vi "VIH Dialog - VI Terminals.vi"(6 "mode (normal)":enum16{"normal", "Enum sel"}(ring), 7 "Called from Master (F)":bool, 10 "Ctrl IDs in":string[](array[string]), 11 "VI Path":path) -> (0 "OK out":bool, 1 "Ctrl Rules":T1[](array[typedef]), 2 "Ctrl IDs out":string[](array[string]), 3 "dup VI Path":path)   [LabVIEW 2014]
doc: "::: VI Helpeks :::\nCopyright (c) 2000-2026 Konstantin Shifershteyn. All rights reserved."
uses:
  _VIH HelpGen.llb/VIH HelpGen Typedef - Cluster - Control Rule.ctl
  _VIH HelpGen.llb/VIH HelpGen Typedef - Enum - Description Mode.ctl
  _VIH HelpGen.llb/VIH HelpGen Typedef - Enum - Default,Enable,Disable.ctl
  _VIH HelpGen.llb/VIH HelpGen Typedef - Cluster - Enum Value Info.ctl
  <vilib>/Utility/miscctls.llb/LVPointTypeDef.ctl
  <vilib>/event_ctls.llb/lveventtype.ctl
  <vilib>/Utility/cursorutil.llb/Set Cursor (Icon Pict).vi
  _VIH Support Library.llb/VIH Utility - APP - Is Value Changed (I32).vi
panel:
  out "Conpane Image":picture caption="Connector Pane Image"
  in  "ConpaneMenuActive":bool
  in  "Ctrl Tree":string[](tree) caption="Control Tree"
  in  "%OK":bool caption="OK"
  in  "%Cancel":bool caption="Cancel"
  # "*) use Context Help for information on the controls"
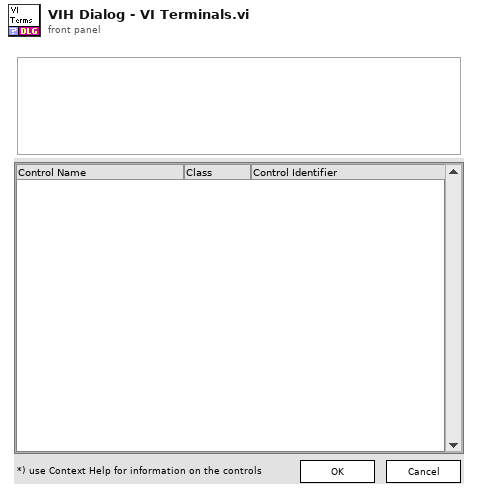
[diagram p1: front panel]
types:
  T1 = typedef "VIH HelpGen Typedef - Cluster - Control Rule.ctl" = cluster{"CtrlID":string, "CustomRule":bool, "DscrMode":T2, "Description":string, "ClusterMembers":T3, "EnumValues":T3, "EnumValDscr":T4[], "CustomName":string}
  T2 = typedef "VIH HelpGen Typedef - Enum - Description Mode.ctl" = enum16{"Default", "Description", "Description1", "Description2", "Custom", "None"}
  T3 = typedef "VIH HelpGen Typedef - Enum - Default,Enable,Disable.ctl" = enum16{"Default", "Enable", "Disable"}
  T4 = typedef "VIH HelpGen Typedef - Cluster - Enum Value Info.ctl" = cluster{"Value":ext, "String":string, "Description":string}
  T5 = typedef "LVPointTypeDef.ctl" = cluster{"Horizontal":i16, "Vertical":i16}
  T6 = typedef "lveventtype.ctl" = enum32{"Null", "Timeout", "Annotation Menu Selection", "Annotation Menu Selection?", "App Instance Close", "App Instance Close?", "Autoscale Range Change", "Bookmark Info Change", "Cell Edit", "Cell Edit?", "Cursor Grab", "Cursor Grab?", "Cursor Menu Selection", "Cursor Menu Selection?", "Cursor Move", "Cursor Release", "Data Change", "Direction Change", "Display State Change", "Drag Ended", "Drag Enter", "Drag Leave", "Drag Over", "Drag Source Update", "Drag Starting", "Drag Starting?", "Drop", "Exec State Change", "Key Down", "Key Down?", "Key Repeat", "Key Repeat?", "Key Up", "Listbox Double Click", "Menu Activation?", "Menu Selection (App)", "Menu Selection? (App)", "Menu Selection (User)", "Mouse Down", "Mouse Down?", "Mouse Enter", "Mouse Leave", "Mouse Move", "Mouse Up", "Mouse Wheel", "NI Security User Change (App)", "Pane Size", "Panel Close", "Panel Close?", "Panel Resize", "Plot Attribute Change", "Scale Range Change", "Shortcut Menu Activation?", "Shortcut Menu Selection (App)", "Shortcut Menu Selection? (App)", "Shortcut Menu Selection (User)", "Tree Double Click", "Tree Drag", "Tree Drag?", "Tree Drop", "Tree Drop?", "Tree Item Close", "Tree Item Close?", "Tree Item Open", "Tree Item Open?", "User Event", "Value Change"}
  T7 = cluster{"Width":i16, "Style":enum32{"Solid", "Dash", "Dot", "DashDot", "DashDotDot"}}
  T8 = typedef "LVPoint32TypeDef.ctl" = cluster{"Horizontal":i32, "Vertical":i32}
  T9 = typedef "LVMouseTypeDef.ctl" = cluster{"Mouse Position":cluster{"X":i32, "Y":i32}, "Mouse Modifiers":cluster{"Button Down":bool, "Shift Mod":bool, "Menu Mod":bool, "Option Mod":bool}}
  T10 = cluster{"Button Down":bool, "Shift Mod":bool, "Menu Mod":bool, "Option Mod":bool}
  T11 = cluster{"Ctrl ID":string, "Conpane Idx":i32, "Bounds":cluster{"X0":i32, "Y0":i32, "X1":i32, "Y1":i32}}[]
  T12 = cluster{"Ctrl ID":string, "Conpane Idx":i32, "Bounds":cluster{"X0":i32, "Y0":i32, "X1":i32, "Y1":i32}}
  T13 = typedef "VIH Project Tree Typedef - Tree Refnum.ctl" = refnum<vi>
  T14 = cluster{"Control Label":string, "Class Name":string, "Indicator":bool, "Error Cluster":bool, "Tree Tag":string, "Control ID":string, "Conpane Idx":i32}
  T15 = typedef "imagedata.ctl" = cluster{"image type":i32, "image depth":i32, "image":u8[], "mask":u8[], "colors":u32[], "Rectangle":cluster{"left":i16, "top":i16, "right":i16, "bottom":i16}}
  T16 = cluster{"left":i16, "top":i16, "right":i16, "bottom":i16}
  T17 = typedef "VIH HelpGen Typedef - Control Terminal Attributes Cluster.ctl" = cluster{"Conpane Idx":i32, "Control":bool, "Wire Rule":enum16{"Invalid Wire Rule", "Required", "Recommended", "Optional", "Dynamic Dispatch"}}
  T18 = cluster{"Control Label":string, "Class Name":string, "Indicator":bool, "Error Cluster":bool, "Tree Tag":string, "Control ID":string, "Conpane Idx":i32}[]
  T19 = typedef "LVBoundsTypeDef.ctl" = cluster{"Width":u32, "Height":u32}
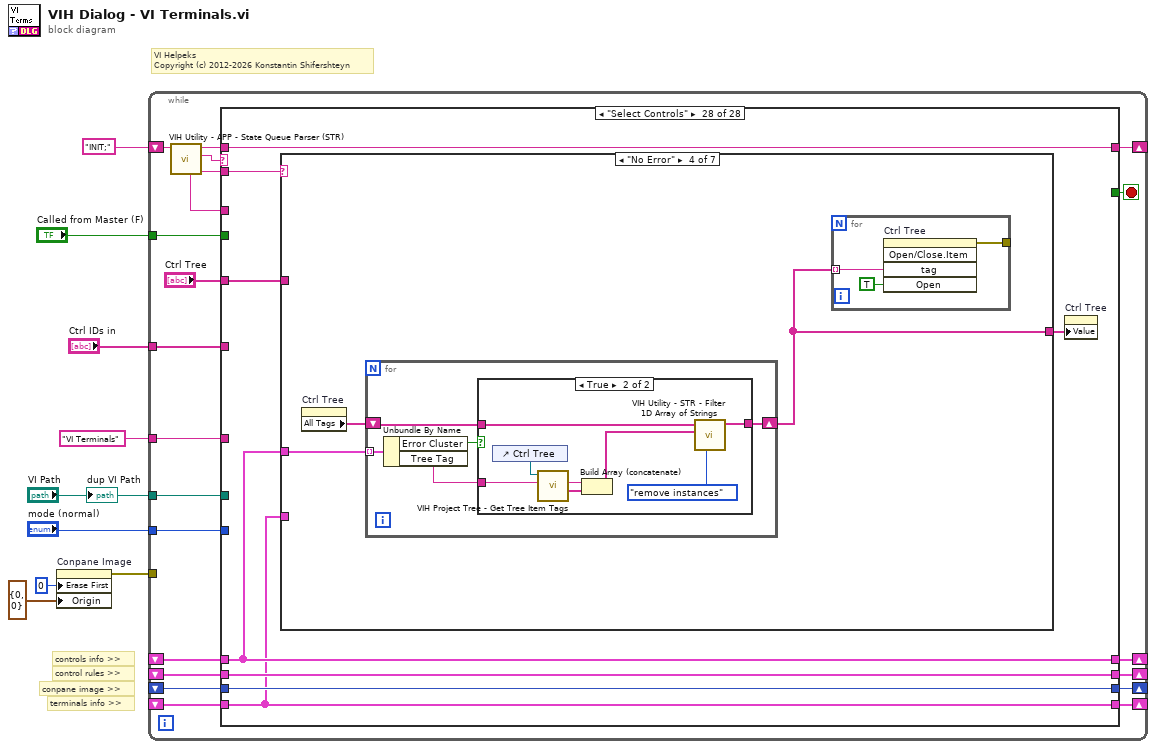
[diagram p0: block diagram]
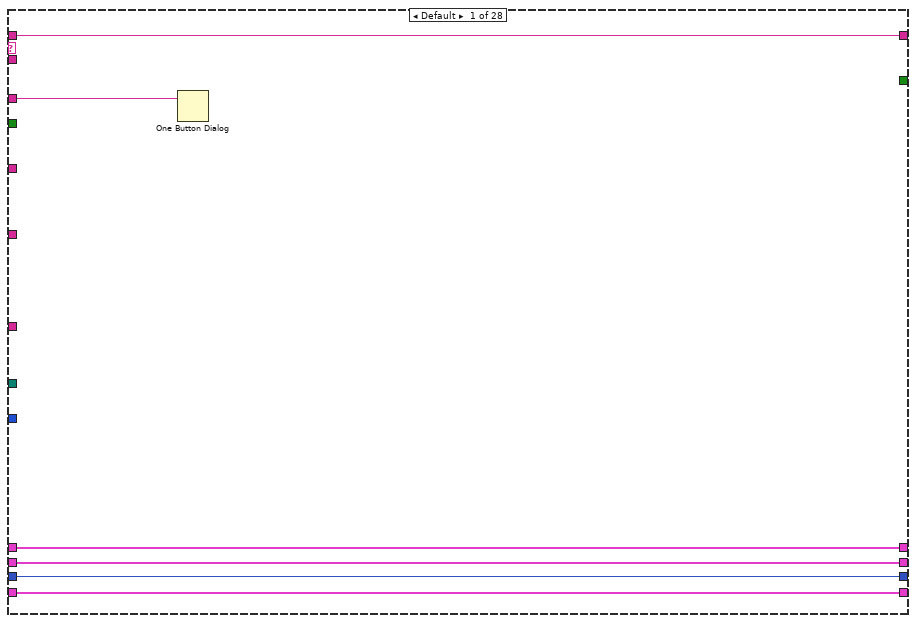
[diagram p2: hidden frame]
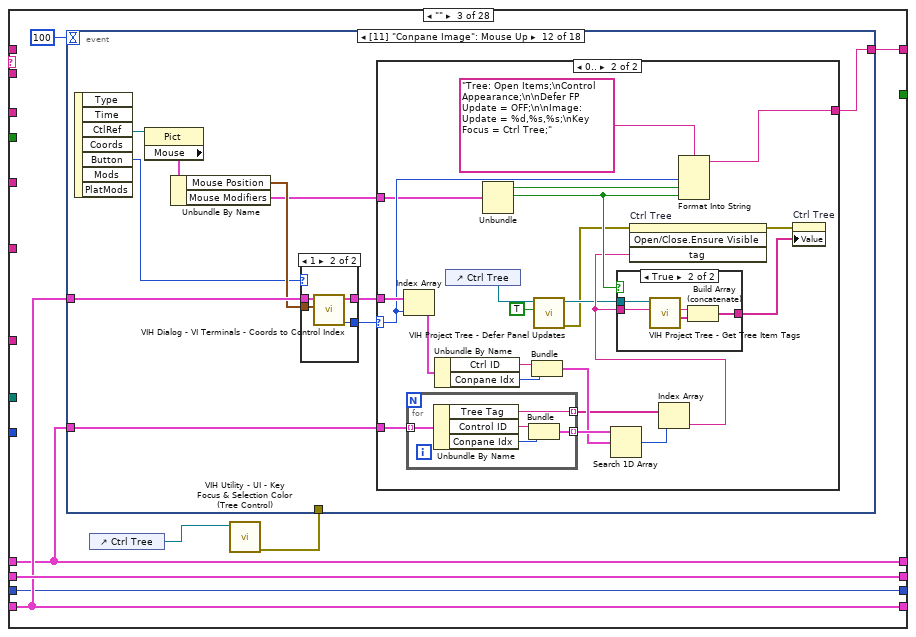
[diagram p4: hidden frame]
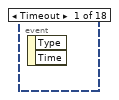
[diagram p5: hidden frame]
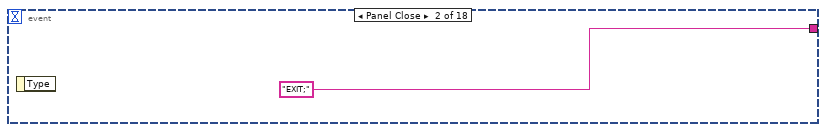
[diagram p6: hidden frame]
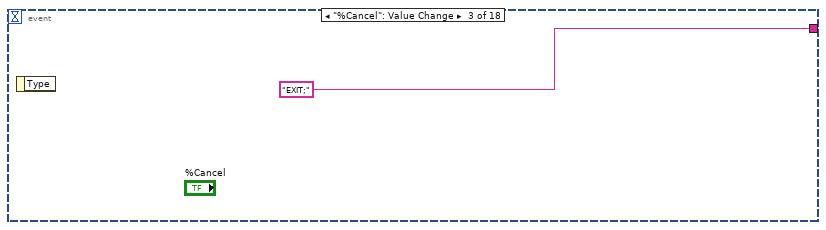
[diagram p7: hidden frame]
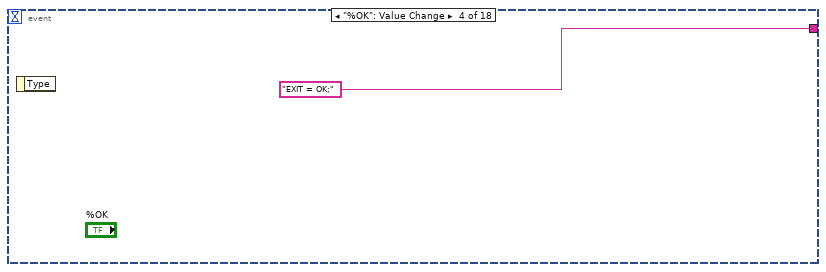
[diagram p8: hidden frame]
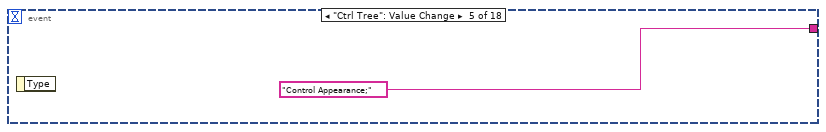
[diagram p9: hidden frame]
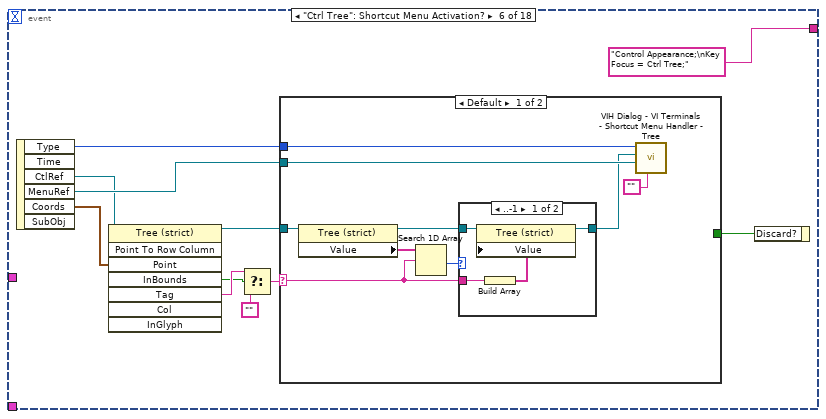
[diagram p10: hidden frame]
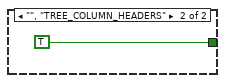
[diagram p12: hidden frame]
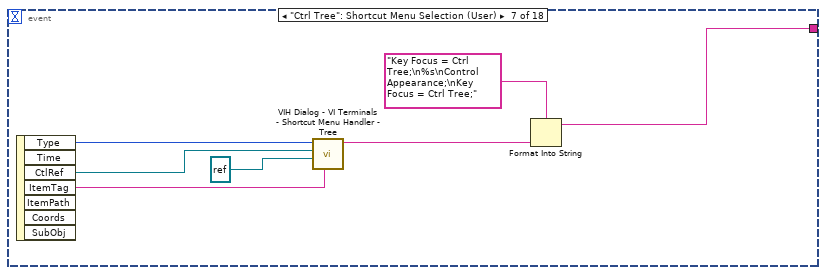
[diagram p13: hidden frame]
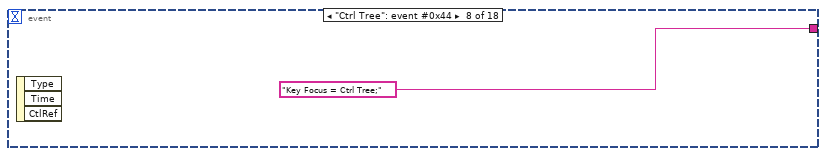
[diagram p14: hidden frame]
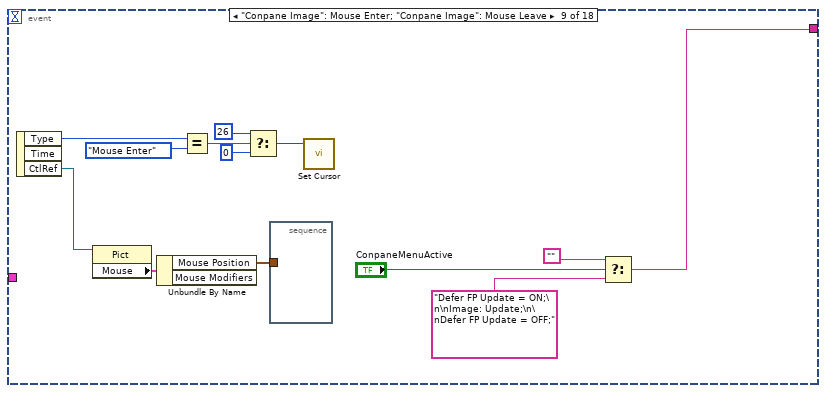
[diagram p15: hidden frame]
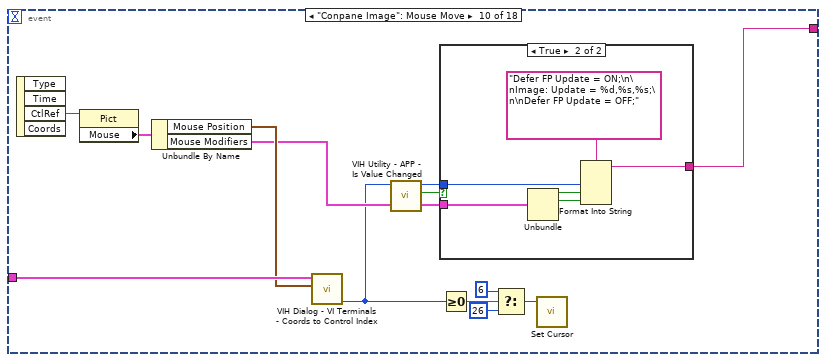
[diagram p16: hidden frame]
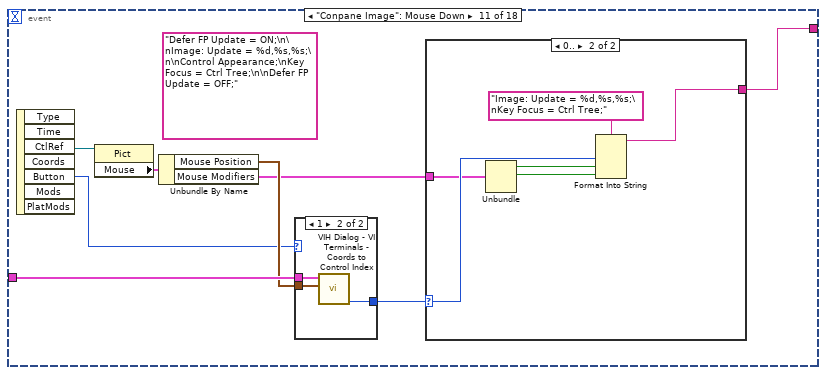
[diagram p18: hidden frame]
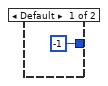
[diagram p19: hidden frame]
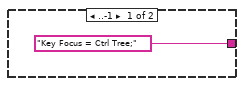
[diagram p20: hidden frame]
diagram:
  # "VI Helpeks\nCopyright (c) 2012-2026 Konstantin Shifershteyn"
  # "terminals info >>"
  # "conpane image >>"
  # "controls info >>"
  # "control rules >>"
  n1 = property on="Conpane Image" class="Pict"("Erase First"=u8 0, "Origin"=T5 {"Horizontal"=0, "Vertical"=0}) -> (error out=w5:errorcluster)  [unwired: 2 in, 1 out]
  n2 = while {
    shift-right: [w27] -> _
    shift-left: "INIT;" -> [w29]
    tunnel: "VI Path" -> [w25]
    shift-right: [w21] -> _
    shift-left: _ -> [w20]
    shift-right: [w19] -> _
    shift-left: _ -> [w18]
    shift-right: [w17] -> _
    shift-left: _ -> [w16]
    tunnel: w5 -> [_]
    tunnel: "Ctrl IDs in" -> [w15]
    tunnel: "mode (normal)" -> [w14]
    tunnel: "Called from Master (F)" -> [w13]
    shift-right: [w12] -> _
    shift-left: _ -> [w11]
    tunnel: "VI Terminals" -> [w10]
    stop <- w22 stop-if-true
    n3 = call "VIH Utility - APP - State Queue Parser (STR).vi"("input queue"=w29) -> ("state parameters"=w24:string, "state"=w30:string, "remained queue"=w28:string, "complete state specifier"=w26:string)  [unwired: 5 in]
    n4 = case shown="\"Select Controls\"" w30 {
      tunnel: w28 -> [w36 w41 _ w286 _ w327 w332 w338 w346 w359 w383 w389 w394 w439 w452 w491 w504 w510 w516 w523 w537 w569 w578 w595 w616 w639 w646 w654]
      tunnel: [w36 w41 w46 w280 "Tree: Reset;\nHALT;" w327 w332 w338 w346 w359 w383 w389 w394 w439 w452 w491 w504 w510 w516 w523 w537 w569 w578 w595 w616 w639 w646 w654] -> w27
      tunnel: w26 -> [w35 _ _ _ _ _ _ _ _ _ _ _ _ _ _ _ _ _ _ _ _ _ _ _ _ _ _ _]
      tunnel: w25 -> [_ _ _ _ _ _ _ _ _ _ _ _ _ w438 _ _ _ _ _ _ _ _ _ _ _ _ _ _]
      tunnel: w24 -> [_ _ _ _ w293 _ _ w337 w345 _ w380 _ _ _ _ _ _ _ _ _ w535 _ _ _ _ _ _ w651]
      tunnel: "Ctrl Tree" -> [_ _ _ _ w292 _ _ _ _ w353 _ _ _ _ _ _ _ _ w512 _ _ _ w581 w598 w609 w635 _ w650]
      tunnel: [_ _ _ _ _ TRUE _ _ _ _ _ _ _ _ _ _ _ _ _ _ _ _ _ _ _ _ _ _] -> w22
      tunnel: [w34 w40 w45 w283 w291 w325 w331 w336 w342 w354 w382 w388 w393 w434 w447 w487 T1[] [] w508 w515 w522 w536 w568 w580 w597 w617 w631 w645 w648] -> w21
      tunnel: w20 -> [w34 w40 w45 w283 w291 w325 w331 w336 w342 w354 w382 w388 w393 _ w447 w487 _ w508 w515 w522 w536 w568 w580 w597 w617 w631 w645 w648]
      tunnel: [w33 w39 w44 w282 w290 w323 w330 w335 w341 w358 w381 w387 w392 w417 w445 w489 w501 w507 w514 w521 w531 w567 w572 w593 w614 w637 w644 w647] -> w19
      tunnel: w18 -> [w33 w39 w44 w282 w290 w323 w330 w335 w341 w358 w381 w387 w392 _ w445 w489 w501 w507 w514 w521 w531 w567 w572 w593 w614 w637 w644 w647]
      tunnel: [w32 w38 w43 w281 w289 w322 w329 w334 w340 w357 w379 w386 w391 w404 w446 w490 w500 w506 w513 w520 w530 w566 w571 w592 w613 w636 w643 w653] -> w17
      tunnel: w16 -> [w32 w38 w43 w281 w289 w322 w329 w334 w340 w357 w379 w386 w391 _ w446 w490 w500 w506 w513 w520 w530 w566 w571 w592 w613 w636 w643 w653]
      tunnel: w15 -> [_ _ _ _ _ _ _ _ _ _ _ _ _ _ w450 _ _ _ _ _ _ _ _ _ _ _ _ _]
      tunnel: w14 -> [_ _ _ w271 _ _ _ _ _ w356 _ _ _ _ _ _ _ _ _ _ _ _ _ _ _ _ _ _]
      tunnel: w13 -> [_ _ _ w273 _ _ _ _ _ w351 _ _ _ _ w448 _ _ _ _ _ _ _ _ _ _ _ _ _]
      tunnel: [w31 w37 w42 w274 w288 w321 w328 w333 w339 w348 w378 w385 w390 w396 w444 w488 w499 w505 w511 w519 w524 w565 w570 w589 w611 w626 w642 w649] -> w12
      tunnel: w11 -> [w31 w37 w42 w274 w288 w321 w328 w333 w339 w348 w378 w385 w390 _ w444 w488 w499 w505 w511 w519 w524 w565 w570 w589 w611 w626 w642 w649]
      tunnel: w10 -> [_ _ _ w268 _ w316 _ _ _ _ _ _ _ _ _ _ _ _ _ _ _ _ _ _ _ _ _ _]
      frame Default {
        n5 = One Button Dialog(message=w35) -> ()  [unwired: 1 in, 1 out]
      }
      frame "#" {
      }
      frame "" {
        n6 = control-ref of="Ctrl Tree"() -> (w48:refnum<vi>)
        n7 = call "VIH Utility - UI - Key Focus & Selection Color (Tree Control).vi"("Tree Refnum"=w48) -> ("error out"=w47:errorcluster)  [unwired: 8 in, 2 out]
        n8 = event shown="[11] \"Conpane Image\": Mouse Up" {
          selector: _ -> [_ _ _ _ _ _ _ _ _ _ _ _ _ _ _ _ _ _]
          dyn-events: _ -> [_ _ _ _ _ _ _ _ _ _ _ _ _ _ _ _ _ _]
          timeout: 100 -> [_ _ _ _ _ _ _ _ _ _ _ _ _ _ _ _ _ _]
          tunnel: w47 -> [_ _ _ _ _ _ _ _ _ _ _ _ _ _ _ _ _ _]
          tunnel: [_ "EXIT;" "EXIT;" "EXIT = OK;" "Control Appearance;" "Control Appearance;\nKey Focus = Ctrl Tree;" w81 "Key Focus = Ctrl Tree;" w91 w109 w125 w145 w208 w236 "Key Focus = Ctrl Tree;" "Image: Update;" "Image: Update;" w260] -> w46
          tunnel: w44 -> [_ _ _ _ _ _ _ _ _ w113 w127 w148 w214 w233 w248 _ _ w261]
          tunnel: w42 -> [_ _ _ _ _ _ _ _ _ _ _ w139 w192 w220 _ _ _ _]
          event Timeout {
            n9 = event-data() -> ()  [unwired: 1 in, 2 out]
          }
          event Panel Close {
            n10 = event-data() -> ()  [unwired: 1 in, 1 out]
          }
          event "%Cancel": Value Change {
            n11 = event-data() -> ()  [unwired: 1 in, 1 out]
          }
          event "%OK": Value Change {
            n12 = event-data() -> ()  [unwired: 1 in, 1 out]
          }
          event "Ctrl Tree": Value Change {
            n13 = event-data() -> ()  [unwired: 1 in, 1 out]
          }
          event "Ctrl Tree": Shortcut Menu Activation? {
            n14 = event-data() -> ("Type"=w57:T6, "CtlRef"=w54:refnum<vi>, "MenuRef"=w56:refnum<k9>, "Coords"=w55:T8)  [unwired: 1 in, 2 out]
            n15 = invoke class="Tree (strict)" method="Point To Row Column"(reference=w54, "Point"=w55) -> (reference out=w63:refnum<vi>, "InBounds"=w59:bool, "Tag"=w60:string)  [unwired: 6 in, 5 out]
            n16 = Select(t=w60, s=w59, f="") -> (s? t:f=w62:string)
            n17 = case shown="Default" w62 {
              selector: w62 -> [w68 _]
              tunnel: w56 -> [w69 _]
              tunnel: [_ TRUE] -> w58
              tunnel: w63 -> [w66 _]
              tunnel: w57 -> [w70 _]
              frame Default {
                n18 = property class="Tree (strict)"(reference=w66) -> (reference out=w71:refnum<vi>, "Value"=w73:string[])  [unwired: 1 in, 1 out]
                n19 = Search 1D Array(1D array=w73, element=w68) -> (index of element=w72:i32)  [unwired: 1 in]
                n20 = case shown="..-1" w72 {
                  tunnel: w71 -> [w77 w78]
                  tunnel: w68 -> [w76 _]
                  tunnel: [w74 w78] -> w65
                  frame ..-1 {
                    n21 = Build Array(w76) -> (w75:string[])
                    n22 = property class="Tree (strict)"(reference=w77, "Value"=w75) -> (reference out=w74:refnum<vi>)  [unwired: 1 in, 1 out]
                  }
                  frame 0.. {
                  }
                }
                n23 = call "VIH Dialog - VI Terminals - Shortcut Menu Handler - Tree.vi"("Menu Tag"="", "MenuRef"=w69, "Terminals Tree"=w65, "Event Type"=w70) -> ()  [unwired: 7 in, 1 out]
              }
              frame "", "TREE_COLUMN_HEADERS" {
              }
            }
            n24 = event-data("Discard?"=w58) -> ()  [unwired: 1 in, 1 out]
          }
          event "Ctrl Tree": Shortcut Menu Selection (User) {
            n25 = event-data() -> ("Type"=w85:T6, "CtlRef"=w84:refnum<vi>, "ItemTag"=w83:string)  [unwired: 1 in, 4 out]
            n26 = call "VIH Dialog - VI Terminals - Shortcut Menu Handler - Tree.vi"("Menu Tag"=w83, "MenuRef"=refnum<k9> refnum, "Terminals Tree"=w84, "Event Type"=w85) -> ("States spec"=w82:string)  [unwired: 7 in]
            n27 = Format Into String(format string="Key Focus = Ctrl Tree;\n%s\nControl Appearance;\nKey Focus = Ctrl Tree;", w82) -> (resulting string=w81:string)  [unwired: 2 in, 1 out]
          }
          event "Ctrl Tree": event #0x44 {
            n28 = event-data() -> ()  [unwired: 1 in, 3 out]
          }
          event "Conpane Image": Mouse Enter; "Conpane Image": Mouse Leave {
            n29 = event-data() -> ("Type"=w100:T6, "CtlRef"=w89:refnum<vi>)  [unwired: 1 in, 1 out]
            n30 = property on="Property Node" class="Pict"(reference=w89) -> ("Mouse"=w90:T9)  [unwired: 1 in, 2 out]
            n31 = Unbundle By Name(w90) -> ("Mouse Position"=w88:cluster{"X":i32, "Y":i32})  [unwired: 1 out]
            n32 = Equal?(x=w100, y=lveventtype."Mouse Enter" ("Type")) -> (x = y?=w98:bool)
            n33 = Select(t=u16 26 ("icon"), s=w98, f=u16 0) -> (s? t:f=w95:u16)
            n34 = stacked-sequence {
              tunnel: w88 -> [_]
              frame #0 {
              }
            }
            n35 = call-poly <vilib>:"Set Cursor.vi"("icon"=w95) -> ()  [unwired: 9 in, 2 out]
            n36 = Select(t="", s="ConpaneMenuActive", f="Defer FP Update = ON;\n\nImage: Update;\n\nDefer FP Update = OFF;") -> (s? t:f=w91:string)
          }
          event "Conpane Image": Mouse Move {
            n37 = event-data() -> ("CtlRef"=w112:refnum<vi>)  [unwired: 1 in, 3 out]
            n38 = property on="Property Node" class="Pict"(reference=w112) -> ("Mouse"=w111:T9)  [unwired: 1 in, 2 out]
            n39 = Unbundle By Name(w111) -> ("Mouse Position"=w110:cluster{"X":i32, "Y":i32}, "Mouse Modifiers"=w106:T10)
            n40 = call "VIH Dialog - VI Terminals - Coords to Control Index.vi"("Coords"=w110, "Controls info"=w113) -> ("Index"=w101:i32)  [unwired: 8 in, 1 out]
            n41 = call-poly "VIH Utility - APP - Is Value Changed.vi"("Value"=w101) -> ("Changed"=w107:bool, "dup Value"=w108:i32)  [unwired: 5 in]
            n42 = case shown="True" w107 {
              tunnel: [_ w118] -> w109
              tunnel: w108 -> [_ w117]
              tunnel: w106 -> [_ w116]
              frame False {
              }
              frame True {
                n43 = Unbundle(w116) -> ("Button Down"=w115:bool, "Shift Mod"=w114:bool)  [unwired: 2 out]
                n44 = Format Into String(format string="Defer FP Update = ON;\n\nImage: Update = %d,%s,%s;\n\nDefer FP Update = OFF;", w117, w115, w114) -> (resulting string=w118:string)  [unwired: 2 in, 1 out]
              }
            }
            n45 = Greater Or Equal To 0?(x=w101) -> (x >= 0?=w105:bool)
            n46 = Select(t=u16 6 ("icon"), s=w105, f=u16 26) -> (s? t:f=w104:u16)
            n47 = call-poly <vilib>:"Set Cursor.vi"("icon"=w104) -> ()  [unwired: 9 in, 2 out]
          }
          event "Conpane Image": Mouse Down {
            (unwired) "Defer FP Update = ON;\n\nImage: Update = %d,%s,%s;\n\nControl Appearance;\nKey Focus = Ctrl Tree;\n\nDefer FP Update = OFF;"
            n48 = event-data() -> ("CtlRef"=w123:refnum<vi>, "Button"=w120:u16)  [unwired: 1 in, 5 out]
            n49 = property on="Property Node" class="Pict"(reference=w123) -> ("Mouse"=w124:T9)  [unwired: 1 in, 2 out]
            n50 = Unbundle By Name(w124) -> ("Mouse Position"=w122:cluster{"X":i32, "Y":i32}, "Mouse Modifiers"=w121:T10)
            n51 = case shown="1" w120 {
              tunnel: w127 -> [_ w131]
              tunnel: [-1 ("Index") w130] -> w126
              tunnel: w122 -> [_ w129]
              frame Default {
              }
              frame 1 {
                n52 = call "VIH Dialog - VI Terminals - Coords to Control Index.vi"("Coords"=w129, "Controls info"=w131) -> ("Index"=w130:i32)  [unwired: 8 in, 1 out]
              }
            }
            n53 = case shown="0.." w126 {
              selector: w126 -> [_ w137]
              tunnel: ["Key Focus = Ctrl Tree;" w136] -> w125
              tunnel: w121 -> [_ w134]
              frame ..-1 {
              }
              frame 0.. {
                n54 = Unbundle(w134) -> ("Button Down"=w133:bool, "Shift Mod"=w135:bool)  [unwired: 2 out]
                n55 = Format Into String(format string="Image: Update = %d,%s,%s;\nKey Focus = Ctrl Tree;", w137, w133, w135) -> (resulting string=w136:string)  [unwired: 2 in, 1 out]
              }
            }
          }
          event "Conpane Image": Mouse Up {
            n56 = event-data() -> ("CtlRef"=w143:refnum<vi>, "Button"=w140:u16)  [unwired: 1 in, 5 out]
            n57 = property on="Property Node" class="Pict"(reference=w143) -> ("Mouse"=w144:T9)  [unwired: 1 in, 2 out]
            n58 = Unbundle By Name(w144) -> ("Mouse Position"=w142:cluster{"X":i32, "Y":i32}, "Mouse Modifiers"=w141:T10)
            n59 = case shown="1" w140 {
              tunnel: w148 -> [w150 w154]
              tunnel: [w150 w153] -> w147
              tunnel: [-1 ("Index") w152] -> w146
              tunnel: w142 -> [_ w151]
              frame 0, Default {
              }
              frame 1 {
                n60 = call "VIH Dialog - VI Terminals - Coords to Control Index.vi"("Coords"=w151, "Controls info"=w154) -> ("Index"=w152:i32, "dup Controls info"=w153:T11)  [unwired: 8 in]
              }
            }
            n61 = case shown="0.." w146 {
              selector: w146 -> [_ w174]
              tunnel: w147 -> [_ w177]
              tunnel: ["Key Focus = Ctrl Tree;" w173] -> w145
              tunnel: w141 -> [_ w172]
              tunnel: w139 -> [_ w167]
              frame ..-1 {
                (unwired) "Image: Update;\nKey Focus = Ctrl Tree;"
              }
              frame 0.. {
                n62 = Index Array(array=w177, index=w174) -> (element=w176:T12)
                n63 = for {
                  tunnel: w167 -> [w182] mode=indexing
                  tunnel: [w180] -> w166 mode=indexing
                  tunnel: [w179] -> w162 mode=indexing
                  n64 = Unbundle By Name(w182) -> ("Tree Tag"=w179:string, "Control ID"=w181:string, "Conpane Idx"=w178:i32)
                  n65 = Bundle("Control ID"=w181, "Conpane Idx"=w178) -> (w180:cluster{"Control ID":string, "Conpane Idx":i32})  [unwired: 1 in]
                }
                n66 = Unbundle By Name(w176) -> ("Ctrl ID"=w165:string, "Conpane Idx"=w164:i32)
                n67 = control-ref of="Ctrl Tree"() -> (w157:refnum<vi>)
                n68 = Unbundle(w172) -> ("Button Down"=w171:bool, "Shift Mod"=w168:bool)  [unwired: 2 out]
                n69 = Bundle("Ctrl ID"=w165, "Conpane Idx"=w164) -> (w163:cluster{"Ctrl ID":string, "Conpane Idx":i32})  [unwired: 1 in]
                n70 = call "VIH Project Tree - Defer Panel Updates.vi"("Defer Panel Updates (F)"=TRUE, "Project Tree"=w157) -> ("error out"=w156:errorcluster, "dup Project Tree"=w158:T13)  [unwired: 7 in, 1 out]
                n71 = Search 1D Array(1D array=w166, element=w163) -> (index of element=w161:i32)  [unwired: 1 in]
                n72 = Index Array(array=w162, index=w161) -> (element=w160:string)
                n73 = case shown="True" w168 {
                  tunnel: [w183 w189] -> w170
                  tunnel: w158 -> [_ w188]
                  tunnel: w160 -> [w184 w187]
                  frame False {
                    n74 = Build Array(w184) -> (w183:string[])
                  }
                  frame True {
                    n75 = call "VIH Project Tree - Get Tree Item Tags.vi"("Parent Item Tag"=w187, "Project Tree"=w188) -> ("Child Item Tags"=w185:string[], "dup Parent Item Tag"=w186:string)  [unwired: 6 in, 2 out]
                    n76 = Build Array (concatenate)(w186, w185) -> (w189:string[])
                  }
                }
                n77 = invoke on="Ctrl Tree" class="Tree (strict)" method="Open/Close.Ensure Visible"(error in=w156, "tag"=w160) -> (error out=w169:errorcluster)  [unwired: 2 in, 3 out]
                n78 = Format Into String(format string="Tree: Open Items;\nControl Appearance;\n\nDefer FP Update = OFF;\n\nImage: Update = %d,%s,%s;\nKey Focus = Ctrl Tree;", w174, w171, w168) -> (resulting string=w173:string)  [unwired: 2 in, 1 out]
                n79 = property on="Ctrl Tree" class="Tree (strict)"(error in=w169, "Value"=w170) -> ()  [unwired: 1 in, 2 out]
              }
            }
          }
          event "Conpane Image": Shortcut Menu Activation? {
            n80 = event-data() -> ("Type"=w211:T6, "CtlRef"=w202:refnum<vi>, "MenuRef"=w209:refnum<k9>, "Coords"=w201:T8)  [unwired: 1 in, 1 out]
            n81 = local write "ConpaneMenuActive"(TRUE ("ConpaneMenuActive")) -> ()
            n82 = call "VIH UI - Convert Pane Coords to Picture Control Coords.vi"("Pane Coords"=w201, "Pict Refnum"=w202) -> ("Picture Coords"=w200:cluster{"Horizontal":i32, "Vertical":i32})  [unwired: 8 in, 1 out]
            n83 = call "VIH Dialog - VI Terminals - Coords to Control Index.vi"("Coords"=w200, "Controls info"=w214) -> ("Index"=w213:i32, "dup Controls info"=w212:T11)  [unwired: 8 in]
            n84 = for {
              tunnel: w192 -> [w218] mode=indexing
              tunnel: [w216] -> w196 mode=indexing
              n85 = Unbundle By Name(w218) -> ("Control ID"=w217:string, "Conpane Idx"=w215:i32)
              n86 = Bundle("Control ID"=w217, "Conpane Idx"=w215) -> (w216:cluster{"Control ID":string, "Conpane Idx":i32})  [unwired: 1 in]
            }
            n87 = Index Array(array=w212, index=w213) -> (element=w191:T12)
            n88 = Unbundle By Name(w191) -> ("Ctrl ID"=w195:string, "Conpane Idx"=w194:i32)
            n89 = Bundle("Ctrl ID"=w195, "Conpane Idx"=w194) -> (w193:cluster{"Ctrl ID":string, "Conpane Idx":i32})  [unwired: 1 in]
            n90 = control-ref of="Ctrl Tree"() -> (w210:refnum<vi>)
            n91 = Search 1D Array(1D array=w196, element=w193) -> (index of element=w190:i32)  [unwired: 1 in]
            n92 = Index Array(array=w192, index=w190) -> (element=w199:T14)
            n93 = Unbundle By Name(w199) -> ("Tree Tag"=w197:string, "Class Name"=w198:string)
            n94 = Format Into String(format string="Image: Update = %d,%s,%s;\nKey Focus = Ctrl Tree;", w213, FALSE, FALSE) -> (resulting string=w208:string)  [unwired: 2 in, 1 out]
            n95 = call "VIH Dialog - VI Terminals - Shortcut Menu Handler - Picture.vi"("Class Name"=w198, "Menu Tag"="", "Tree Item Tag"=w197, "MenuRef"=w209, "Terminals Tree"=w210, "Event Type"=w211) -> ()  [unwired: 5 in, 1 out]
            n96 = event-data() -> ()  [unwired: 2 in, 1 out]
          }
          event "Conpane Image": Shortcut Menu Selection (User) {
            n97 = event-data() -> ("Type"=w241:T6, "CtlRef"=w229:refnum<vi>, "ItemTag"=w234:string, "Coords"=w230:T8)  [unwired: 1 in, 3 out]
            n98 = call "VIH UI - Convert Pane Coords to Picture Control Coords.vi"("Pane Coords"=w230, "Pict Refnum"=w229) -> ("Picture Coords"=w228:cluster{"Horizontal":i32, "Vertical":i32})  [unwired: 8 in, 1 out]
            n99 = control-ref of="Ctrl Tree"() -> (w240:refnum<vi>)
            n100 = call "VIH Dialog - VI Terminals - Coords to Control Index.vi"("Coords"=w228, "Controls info"=w233) -> ("Index"=w231:i32, "dup Controls info"=w232:T11)  [unwired: 8 in]
            n101 = for {
              tunnel: w220 -> [w245] mode=indexing
              tunnel: [w243] -> w225 mode=indexing
              n102 = Unbundle By Name(w245) -> ("Control ID"=w244:string, "Conpane Idx"=w242:i32)
              n103 = Bundle("Control ID"=w244, "Conpane Idx"=w242) -> (w243:cluster{"Control ID":string, "Conpane Idx":i32})  [unwired: 1 in]
            }
            n104 = Index Array(array=w232, index=w231) -> (element=w221:T12)
            n105 = Unbundle By Name(w221) -> ("Ctrl ID"=w224:string, "Conpane Idx"=w223:i32)
            n106 = Bundle("Ctrl ID"=w224, "Conpane Idx"=w223) -> (w222:cluster{"Ctrl ID":string, "Conpane Idx":i32})  [unwired: 1 in]
            n107 = Search 1D Array(1D array=w225, element=w222) -> (index of element=w219:i32)  [unwired: 1 in]
            n108 = Index Array(array=w220, index=w219) -> (element=w227:T14)
            n109 = Unbundle By Name(w227) -> ("Tree Tag"=w226:string)
            n110 = call "VIH Dialog - VI Terminals - Shortcut Menu Handler - Picture.vi"("Menu Tag"=w234, "Tree Item Tag"=w226, "MenuRef"=refnum<k9> refnum, "Terminals Tree"=w240, "Event Type"=w241) -> ("States spec"=w237:string)  [unwired: 6 in]
            n111 = local write "ConpaneMenuActive"(FALSE ("ConpaneMenuActive")) -> ()
            n112 = Format Into String(format string="Key Focus = Ctrl Tree;\n\n%s\nControl Appearance;\n\nDefer FP Update = OFF;\nKey Focus = Ctrl Tree;", w237) -> (resulting string=w236:string)  [unwired: 2 in, 1 out]
          }
          event "Conpane Image": event #0x44 {
            (unwired) "Image: Update;\nKey Focus = Ctrl Tree;"
            n113 = event-data() -> ("CtlRef"=w249:refnum<vi>)  [unwired: 1 in, 2 out]
            n114 = property on="Property Node" class="Pict"(reference=w249) -> ("Mouse"=w250:T9)  [unwired: 1 in, 2 out]
            n115 = Unbundle By Name(w250) -> ("Mouse Position"=w247:cluster{"X":i32, "Y":i32})  [unwired: 1 out]
            n116 = local write "ConpaneMenuActive"(FALSE ("ConpaneMenuActive")) -> ()
            n117 = call "VIH Dialog - VI Terminals - Coords to Control Index.vi"("Coords"=w247, "Controls info"=w248) -> ("Index"=w246:i32)  [unwired: 8 in, 1 out]
            n118 = stacked-sequence {
              tunnel: w246 -> [_]
              frame #0 {
              }
            }
          }
          event Mouse Enter {
            n119 = event-data() -> ()  [unwired: 1 in, 3 out]
          }
          event Mouse Down {
            n120 = event-data() -> ()  [unwired: 1 in, 7 out]
          }
          event Key Down; Key Up {
            (unwired) "Image: Update = %d,%s,%s;\n\nControl Appearance;\nKey Focus = Ctrl Tree;"
            n121 = event-data() -> ()  [unwired: 1 in, 7 out]
            n122 = property on="Conpane Image" class="Pict"() -> ("Mouse"=w259:T9)  [unwired: 2 in, 2 out]
            n123 = Unbundle By Name(w259) -> ("Mouse Position"=w258:cluster{"X":i32, "Y":i32}, "Mouse Modifiers"=w257:T10)
            n124 = call "VIH Dialog - VI Terminals - Coords to Control Index.vi"("Coords"=w258, "Controls info"=w261) -> ("Index"=w256:i32)  [unwired: 8 in, 1 out]
            n125 = case shown="0.." 0 ("Index") {
              tunnel: [_ w266] -> w260
              tunnel: w257 -> [_ w264]
              tunnel: w256 -> [_ w262]
              frame ..-1 {
              }
              frame 0.. {
                n126 = Unbundle(w264) -> ("Button Down"=w263:bool, "Shift Mod"=w265:bool)  [unwired: 2 out]
                n127 = Format Into String(format string="Image: Update = %d,%s,%s;", w262, w263, w265) -> (resulting string=w266:string)  [unwired: 2 in, 1 out]
              }
            }
          }
        }
      }
      frame "INIT" {
        n128 = case shown="\"Enum sel\"" w271 {
          tunnel: [_ " - Select Enum or Ring Control"] -> w270
          frame "normal" {
          }
          frame "Enum sel" {
          }
        }
        n129 = Not(x=w273) -> (.not. x?=w272:bool)
        n130 = Select(t="Close", s=w273, f="Cancel") -> (s? t:f=w277:string)
        n131 = property on="%OK" class="Bool"("Visible"=w272) -> ()  [unwired: 2 in, 2 out]
        n132 = Initialize Array(w277, 4 ("dimension size")) -> (w275:string[])
        n133 = property on="%Cancel" class="Bool"("Strings [4]"=w275) -> ()  [unwired: 2 in, 2 out]
        n134 = Concatenate Strings(w268, w270) -> (w269:string)
        n135 = property class="VI"("Front Panel.Title"=w269) -> ()  [unwired: 2 in, 2 out]
        n136 = property on="Ctrl Tree" class="Tree (strict)"("Value"=string[] [] ("Item Names")) -> ()  [unwired: 2 in, 2 out]
        n137 = Concatenate Strings("Set Busy = ON;\n\nTree: Reset;\nTree: Message;\n\nOptTerminals Attention;\n\nDefer FP Update = ON;\n\nTree: Reset;\nTree: Build;\nTree: Preset Value;\nTree: Disable Items;\n\nImage: Update;\n\nControl Appearance;\n\nKey Focus = Ctrl Tree;\n\nDefer FP Update = OFF;\n\nSet Busy = OFF;", w286) -> (w280:string)
      }
      frame "EXIT" {
        n138 = case shown="\"OK\"" w293 {
          tunnel: [_ TRUE] -> w296
          tunnel: [_ w298] -> w295
          tunnel: w292 -> [_ w304]
          tunnel: [_ w303] -> w294
          tunnel: w291 -> [_ w301]
          tunnel: w288 -> [_ w300]
          frame Default {
          }
          frame "OK" {
            n139 = for {
              tunnel: w300 -> [w308] mode=indexing
              tunnel: [w307] -> w302 mode=indexing
              tunnel: [w306] -> w299 mode=indexing
              n140 = Unbundle By Name(w308) -> ("Tree Tag"=w307:string, "Control ID"=w306:string)
            }
            n141 = for {
              tunnel: w304 -> [w314] mode=indexing
              tunnel: [w312] -> w303 mode=indexing
              tunnel: w302 -> [w315]
              tunnel: w301 -> [w313]
              tunnel: w299 -> [w310]
              tunnel: [w309] -> w298 mode=indexing
              n142 = Search 1D Array(1D array=w315, element=w314) -> (index of element=w311:i32)  [unwired: 1 in]
              n143 = Index Array(array=w313, index=w311) -> (element=w312:T1)
              n144 = Index Array(array=w310, index=w311) -> (element=w309:string)
            }
          }
        }
        "OK out" <- w296
        "Ctrl IDs out" <- w295
        "Ctrl Rules" <- w294
      }
      frame "HALT" {
        n145 = property class="VI"("Front Panel.Title"=w316) -> ()  [unwired: 2 in, 2 out]
        n146 = Initialize Array("Cancel", 4 ("dimension size")) -> (w317:string[])
        n147 = property on="%Cancel" class="Bool"("Strings [4]"=w317) -> ()  [unwired: 2 in, 2 out]
        n148 = property on="%OK" class="Bool"("Visible"=TRUE) -> ()  [unwired: 2 in, 2 out]
        n149 = property on="Splitter 3" class="Splitter"("Locked"=FALSE ("Splitter Position Locked")) -> ()  [unwired: 2 in, 2 out]
      }
      frame "--------------------------------------- 1" {
      }
      frame "Set Busy" {
        n150 = case shown="\"ON\"" w337 {
          frame "OFF", Default {
            n151 = call <vilib>:"Unset Busy.vi"() -> ()  [unwired: 11 in, 1 out]
          }
          frame "ON" {
            n152 = call <vilib>:"Set Busy.vi"() -> ()  [unwired: 10 in, 2 out]
          }
        }
      }
      frame "Defer FP Update" {
        n153 = case shown="\"ON\"" w345 {
          tunnel: [_ TRUE] -> w343
          frame "OFF", Default {
          }
          frame "ON" {
          }
        }
        n154 = property class="VI"() -> ("Front Panel"=w344:refnum<vi>)  [unwired: 2 in, 2 out]
        n155 = property class="Pnl"(reference=w344, "Defer Panel Updates"=w343) -> ()  [unwired: 1 in, 2 out]
      }
      frame "Control Appearance" {
        n156 = Array Size(array=w353) -> (size(s)=w355:i32)
        n157 = case shown="\"Enum sel\"" w356 {
          tunnel: w355 -> [w360 w365]
          tunnel: w354 -> [_ w364]
          tunnel: w353 -> [_ w363]
          tunnel: [w361 w362] -> w350
          frame "normal" {
            n158 = Less Or Equal To 0?(x=w360) -> (x <= 0?=w361:bool)
          }
          frame "Enum sel" {
            n159 = case shown="1" w365 {
              tunnel: w364 -> [_ w370 _]
              tunnel: w363 -> [_ w374 _]
              tunnel: [TRUE w367 TRUE ("empty?")] -> w362
              frame ..0 {
              }
              frame 1 {
                n160 = for {
                  tunnel: w370 -> [w376] mode=indexing
                  tunnel: [w375] -> w373 mode=indexing
                  n161 = Unbundle By Name(w376) -> ("CtrlID"=w375:string)
                }
                n162 = Index Array(array=w374) -> (element=w372:string)  [unwired: 1 in]
                n163 = Search 1D Array(1D array=w373, element=w372) -> (index of element=w371:i32)  [unwired: 1 in]
                n164 = Index Array(array=w370, index=w371) -> (element=w369:T1)
                n165 = Unbundle By Name(w369) -> ("EnumValDscr"=w368:T4[])
                n166 = Empty Array?(array=w368) -> (empty?=w367:bool)
              }
              frame 2.. {
              }
            }
          }
        }
        n167 = Or(x=w351, y=w350) -> (x .or. y?=w349:bool)
        n168 = call "VIH Utility - UI - Boolean to Control Disable Status.vi"("Status in"=w349) -> ("Control Disable if True"=w352:u8)  [unwired: 3 in, 1 out]
        n169 = property on="%OK" class="Bool"("DisabledEnum"=w352) -> ()  [unwired: 2 in, 2 out]
      }
      frame "Key Focus" {
        n170 = case shown="\"Ctrl Tree\"" w380 {
          frame Default {
          }
          frame "Ctrl Tree" {
            n171 = property on="Ctrl Tree" class="Tree (strict)"("Key Focus"=TRUE) -> ()  [unwired: 2 in, 2 out]
          }
        }
      }
      frame "OptTerminals Attention" {
        n172 = disable-structure shown="Disabled" {
          frame Disabled {
            n173 = call "VIH Dialog - Allow_Optional_Terminals in Context Help.vi"() -> ()  [unwired: 11 in, 1 out]
          }
          frame Enabled {
          }
        }
      }
      frame "--------------------------------------- 2" {
      }
      frame "Tree: Build" {
        n174 = call "VIH HelpGen - Open VI Reference.vi"("Enable Conpane Image Check (T)"=TRUE, "Force use wrapper (F)"=TRUE, "VI Path"=w438) -> ("error out"=w425:errorcluster, "Conpane Image"=w403:T15, "Original VI Name"=w426:string, "VI Reference"=w427:refnum<vi>)  [unwired: 5 in]
        n175 = call "VIH Dialog - VI Terminals - Conpane Image.vi"("error in"=w425, "Conpane Image"=w403, "Original VI Name"=w426, "VI Reference"=w427) -> ("error out"=w424:errorcluster, "Rectangle"=w402:T16, "image"=w404:picture, "dup VI Reference"=w423:refnum<vi>)  [unwired: 4 in]
        n176 = Unbundle(w402) -> ("left"=w400:i16, "top"=w401:i16)  [unwired: 2 out]
        n177 = call "VIH HelpGen - Get VI Conpane Control Refnums.vi"("Sort terminals (T)"=TRUE, "error in"=w424, "VI Reference"=w423) -> ("error out"=w420:errorcluster, "Ctrl Attributes"=w397:T17[], "Conpane Ctrl Refnums"=w416:refnum<vi>[], "dup VI Reference"=w398:refnum<vi>)  [unwired: 5 in]
        n178 = call <vilib>:"Picture to Pixmap.vi"("depth"=24, "picture"=w404) -> ("image data"=w419:T15)  [unwired: 8 in, 1 out]
        n179 = Bundle("top"=w401, "left"=w400) -> (w399:cluster{"top":i16, "left":i16})  [unwired: 1 in]
        n180 = control-ref of="Ctrl Tree"() -> (w432:refnum<vi>)
        n181 = call "VIH HelpGen - Image - Find Ctrl Area in Conpane Picture.vi"("Conpane Image Data"=w419, "error in"=w420, "Top Left"=w399, "Ctrl Attributes"=w397, "Conpane Ctrl Refnums"=w416) -> ("error out"=w421:errorcluster, "Terminals Info"=w417:T11, "dup Conpane Ctrl Refnums"=w415:refnum<vi>[])  [unwired: 2 in, 2 out]
        n182 = call "VIH Dialog - VI Terminals - Build Control Tree.vi"("Ctrl Attributes"=w397, "error in"=w421, "Tree Refnum"=w432, "Ctrl Refnums"=w415) -> ("error out"=w433:errorcluster, "Control Rules"=w434:T1[], "Controls Info"=w396:T18, "dup Ctrl Refnums"=w435:refnum<vi>[])  [unwired: 4 in]
        n183 = Close Reference(reference=w435, error in (no error)=w433) -> (error out=w422:errorcluster)
        n184 = Unbundle By Name(w402) -> ("bottom"=w431:i16)
        n185 = property on="Conpane Image" class="Pict"() -> ("Bounds"=w414:T19, "Draw Area Size"=w413:T19)  [unwired: 2 in, 2 out]
        n186 = call "VIH HelpGen - Close VI Reference.vi"("error in"=w422, "VI Reference"=w398) -> ("error out"=w436:errorcluster)  [unwired: 9 in]
        n187 = To Long Integer(number=w431) -> (32bit integer=w405:i32)
        n188 = Unbundle By Name(w414) -> ("Height"=w409:u32)
        n189 = Unbundle By Name(w413) -> ("Height"=w408:u32)
        n190 = call <vilib>:"Simple Error Handler.vi"("error in (no error)"=w436) -> ()  [unwired: 4 in, 5 out]
        n191 = Add(x=w405, y=5) -> (x+y=w410:i32)
        n192 = To Long Integer(number=w409) -> (32bit integer=w412:i32)
        n193 = To Long Integer(number=w408) -> (32bit integer=w411:i32)
        n194 = Subtract(x=w412, y=w411) -> (x-y=w407:i32)
        n195 = Add(x=w410, y=w407) -> (x+y=w406:i32)
        n196 = Max & Min(x=50 ("Splitter Position"), y=w406) -> (max(x,y)=w428:i32)  [unwired: 1 out]
        n197 = stacked-sequence {
          tunnel: w428 -> [w441]
          frame #0 {
            n198 = property on="Splitter 3" class="Splitter"("Locked"=FALSE ("Splitter Position Locked"), "Position"=w441, "Locked"=TRUE ("Splitter Position Locked")) -> ()  [unwired: 2 in, 2 out]
          }
        }
      }
      frame "Tree: Preset Value" {
        n199 = Empty Array?(array=w450) -> (empty?=w451:bool)
        n200 = case shown="False" w451 {
          tunnel: w450 -> [w461 _]
          tunnel: [w453 w479] -> w449
          tunnel: w448 -> [_ w480]
          tunnel: w444 -> [w460 w481]
          frame False {
            # "a VI might have controls with non-unique names"
            n201 = Array Size(array=w460) -> (size(s)=w459:i32)
            n202 = Initialize Array("", w459) -> (w458:string[])
            n203 = for {
              tunnel: w460 -> [w471] mode=indexing
              tunnel: w461 -> [w469]
              shift-right: [w467] -> w455
              shift-left: w458 -> [w468]
              shift-right: [w466] -> w454
              shift-left: 0 -> [w465]
              n204 = Unbundle By Name(w471) -> ("Tree Tag"=w464:string, "Control ID"=w470:string)
              n205 = Search 1D Array(1D array=w469, element=w470) -> (index of element=w463:i32)  [unwired: 1 in]
              n206 = case shown="0.." w463 {
                tunnel: w468 -> [w473 w478]
                tunnel: [w473 w477] -> w467
                tunnel: [w472 w476] -> w466
                tunnel: w465 -> [w472 w475]
                tunnel: w464 -> [_ w474]
                frame ..-1 {
                }
                frame 0.. {
                  n207 = Replace Array Subset(array=w478, new element=w474, index=w475) -> (w477:string[])
                  n208 = Increment(x=w475) -> (x+1=w476:i32)
                }
              }
            }
            n209 = Reshape Array(w455, w454) -> (w453:string[])
            n210 = Index Array(array=w453) -> (element=w462:string)  [unwired: 1 in]
            n211 = invoke on="Ctrl Tree" class="Tree (strict)" method="Open/Close.Ensure Visible"("tag"=w462) -> ()  [unwired: 3 in, 4 out]
          }
          frame True {
            n212 = case shown="False" w480 {
              tunnel: w481 -> [w483 _]
              tunnel: [w482 _] -> w479
              frame False {
                n213 = for {
                  tunnel: w483 -> [w485] mode=indexing
                  tunnel: [w484] -> w482 mode=indexing
                  n214 = Unbundle By Name(w485) -> ("Tree Tag"=w484:string)
                }
              }
              frame True {
              }
            }
          }
        }
        n215 = property on="Ctrl Tree" class="Tree (strict)"("Value"=w449) -> ()  [unwired: 2 in, 2 out]
      }
      frame "Tree: Disable Items" {
        n216 = case shown="\"Enum sel\"" enum16{"normal", "Enum sel"}."normal" ("mode (normal)") {
          tunnel: w488 -> [_ w492]
          frame "normal" {
          }
          frame "Enum sel" {
            n217 = for {
              tunnel: w492 -> [w495] mode=indexing
              n218 = Unbundle By Name(w495) -> ("Class Name"=w494:string, "Tree Tag"=w493:string)
              n219 = case shown="Default" w494 {
                tunnel: w493 -> [_ w497]
                frame "Enum", "Ring" {
                }
                frame Default {
                  n220 = property on="Ctrl Tree" class="Tree (strict)"("Active Item Tag"=w497, "Disabled?"=TRUE ("Active Item:Disabled?")) -> ()  [unwired: 2 in, 2 out]
                }
              }
            }
          }
        }
      }
      frame "Tree: Reset" {
        n221 = invoke on="Ctrl Tree" class="Tree (strict)" method="Edit Tree Items.Delete"() -> (error out=w503:errorcluster)  [unwired: 5 in, 4 out]
        n222 = property on="Conpane Image" class="Pict"("Erase First"=u8 1) -> ()  [unwired: 2 in, 2 out]
        n223 = invoke on="Ctrl Tree" class="Tree (strict)" method="Custom Item Symbols.Revert Symbols"(error in=w503) -> ()  [unwired: 2 in, 3 out]
      }
      frame "Tree: Message" {
        n224 = invoke on="Ctrl Tree" class="Tree (strict)" method="Edit Tree Items.Add Item to End"("Left Cell"="Collecting information..." ("Left Cell String")) -> ()  [unwired: 7 in, 8 out]
      }
      frame "Tree: Open Items" {
        n225 = for {
          tunnel: w512 -> [w518] mode=indexing
          n226 = invoke on="Ctrl Tree" class="Tree (strict)" method="Open/Close.Item"("tag"=w518, "Open"=TRUE) -> ()  [unwired: 3 in, 5 out]
        }
      }
      frame "--------------------------------------- 3" {
      }
      frame "Image: Update" {
        w527 = FALSE
        n227 = Scan From String(format string="%d,%[^,],%[^,]", input string=w535, default 1=-1 ("default value 1"), default 2=w527, default 3=w527) -> (remaining string=w528:string, output 1=w532:i32, output 2=w526:bool, output 3=w525:bool)  [unwired: 2 in, 2 out]
        n228 = case shown="0.." w532 {
          selector: w532 -> [_ w555]
          tunnel: w531 -> [_ w554]
          tunnel: w530 -> [w538 w553]
          tunnel: [w538 w551] -> w529
          tunnel: w528 -> [_ _]
          tunnel: w526 -> [_ w545]
          tunnel: w525 -> [_ w542]
          frame ..-1 {
          }
          frame 0.. {
            (unwired) u32 255 ("color(black)")
            (unwired) u32 16711680 ("color(black)")
            n229 = Index Array(array=w554, index=w555) -> (element=w552:T12)
            n230 = Unbundle By Name(w552) -> ("Bounds"=w550:cluster{"X0":i32, "Y0":i32, "X1":i32, "Y1":i32})
            n231 = Select(t=i16 2, s=w542, f=i16 1 ("Width")) -> (s? t:f=w539:i16)
            n232 = Bundle By Name(cluster=T7 {"Width"=1, "Style"=enum."Solid"} ("pen"), "Width"=w539) -> (w543:T7)
            n233 = in-place {
              n234 = in-place-cluster #1(w550) -> ("X0"=w564:i32, "Y0"=w559:i32, "X1"=w563:i32, "Y1"=w560:i32)
              n235 = Decrement(x=w559) -> (x-1=w558:i32)
              n236 = Increment(x=w560) -> (x+1=w557:i32)
              n237 = Decrement(x=w564) -> (x-1=w556:i32)
              n238 = Decrement(x=w556) -> (x-1=w562:i32)
              n239 = Increment(x=w563) -> (x+1=w561:i32)
              n240 = in-place-cluster #1("X0"=w562, "Y0"=w558, "X1"=w561, "Y1"=w557) -> (w549:cluster{"X0":i32, "Y0":i32, "X1":i32, "Y1":i32})
            }
            n241 = Select(t=u32 16711680 ("color(black)"), s=w545, f=u32 255 ("color(black)")) -> (s? t:f=w546:u32)
            n242 = call <vilib>:"Draw Rect.vi"("picture"=w553, "rect"=w549, "color(black)"=w546, "pen"=w543) -> ("new picture"=w551:picture)  [unwired: 5 in]
          }
        }
        "Conpane Image" <- w529
      }
      frame "--------------------------------------- 4" {
      }
      frame "Copy to CB: Controls" {
        n243 = for {
          tunnel: w570 -> [w583] mode=indexing
          tunnel: [w582] -> w579 mode=indexing
          n244 = Unbundle By Name(w583) -> ("Tree Tag"=w582:string)
        }
        n245 = for {
          tunnel: w581 -> [w587] mode=indexing
          tunnel: [w584] -> w577 mode=indexing
          tunnel: w579 -> [w588]
          tunnel: w580 -> [w585]
          n246 = Search 1D Array(1D array=w588, element=w587) -> (index of element=w586:i32)  [unwired: 1 in]
          n247 = Index Array(array=w585, index=w586) -> (element=w584:T1)
        }
        n248 = call "VIH XML - Control Rules to-from XML String.vi"("cmd (check)"=enum16{"check", "parse", "format"}."format", "Control Rules in"=w577) -> ("error out"=w574:errorcluster, "XML out"=w575:string)  [unwired: 6 in, 2 out]
        n249 = invoke class="App" method="Clipboard.Write"(error in=w574, "Param 0"=w575) -> (error out=w573:errorcluster)  [unwired: 2 in, 3 out]
        n250 = call <vilib>:"Simple Error Handler.vi"("error in (no error)"=w573) -> ()  [unwired: 4 in, 5 out]
      }
      frame "Copy to CB: Control Names" {
        n251 = for {
          tunnel: w589 -> [w600] mode=indexing
          tunnel: [w599] -> w596 mode=indexing
          n252 = Unbundle By Name(w600) -> ("Tree Tag"=w599:string)
        }
        n253 = for {
          tunnel: w598 -> [w605] mode=indexing
          tunnel: [w601] -> w591 mode=indexing
          tunnel: w596 -> [w606]
          tunnel: w589 -> [w603]
          n254 = Search 1D Array(1D array=w606, element=w605) -> (index of element=w604:i32)  [unwired: 1 in]
          n255 = Index Array(array=w603, index=w604) -> (element=w602:T14)
          n256 = Unbundle By Name(w602) -> ("Control Label"=w601:string)
        }
        n257 = call "VIH Utility - STR - String from 1D Str Array.vi"("Array in"=w591) -> ("String out"=w590:string)  [unwired: 6 in]
        n258 = invoke class="App" method="Clipboard.Write"("Param 0"=w590) -> (error out=w594:errorcluster)  [unwired: 3 in, 3 out]
        n259 = call <vilib>:"Simple Error Handler.vi"("error in (no error)"=w594) -> ()  [unwired: 4 in, 5 out]
      }
      frame "Copy to CB: Control IDs" {
        n260 = for {
          tunnel: w611 -> [w625] mode=indexing
          tunnel: [w624] -> w610 mode=indexing
          tunnel: [w623] -> w608 mode=indexing
          n261 = Unbundle By Name(w625) -> ("Tree Tag"=w624:string, "Control ID"=w623:string)
        }
        n262 = for {
          tunnel: w610 -> [w622]
          tunnel: w609 -> [w621] mode=indexing
          tunnel: w608 -> [w619]
          tunnel: [w618] -> w607 mode=indexing
          n263 = Search 1D Array(1D array=w622, element=w621) -> (index of element=w620:i32)  [unwired: 1 in]
          n264 = Index Array(array=w619, index=w620) -> (element=w618:string)
        }
        n265 = call "VIH Utility - STR - String from 1D Str Array.vi"("Array in"=w607) -> ("String out"=w612:string)  [unwired: 6 in]
        n266 = invoke class="App" method="Clipboard.Write"("Param 0"=w612) -> (error out=w615:errorcluster)  [unwired: 3 in, 3 out]
        n267 = call <vilib>:"Simple Error Handler.vi"("error in (no error)"=w615) -> ()  [unwired: 4 in, 5 out]
      }
      frame "Copy to CB: Enum Values" {
        n268 = for {
          tunnel: w626 -> [w641] mode=indexing
          tunnel: [w640] -> w633 mode=indexing
          n269 = Unbundle By Name(w641) -> ("Tree Tag"=w640:string)
        }
        n270 = Index Array(array=w635) -> (element=w632:string)  [unwired: 1 in]
        n271 = Search 1D Array(1D array=w633, element=w632) -> (index of element=w634:i32)  [unwired: 1 in]
        n272 = Index Array(array=w631, index=w634) -> (element=w630:T1)
        n273 = Unbundle By Name(w630) -> ("EnumValDscr"=w629:T4[])
        n274 = call "VIH XML - Enum Values to-from XML String.vi"("cmd (check)"=enum16{"check", "parse", "format"}."format", "Enum Values in"=w629) -> ("XML out"=w627:string)  [unwired: 6 in, 3 out]
        n275 = invoke class="App" method="Clipboard.Write"("Param 0"=w627) -> (error out=w638:errorcluster)  [unwired: 3 in, 3 out]
        n276 = call <vilib>:"Simple Error Handler.vi"("error in (no error)"=w638) -> ()  [unwired: 4 in, 5 out]
      }
      frame "--------------------------------------- 5" {
      }
      frame "Select Controls" {
        n277 = case shown="\"No Error\"" w651 {
          tunnel: [w655 w658 w659 w687 w708 w726 w741] -> w652
          tunnel: w650 -> [w655 _ _ _ _ _ w740]
          tunnel: w649 -> [_ _ w664 w688 w709 w727 _]
          tunnel: w647 -> [_ _ w668 _ _ _ _]
          frame Default {
          }
          frame "ALL" {
            n278 = invoke on="Ctrl Tree" class="Tree (strict)" method="Open/Close.Open/Close All"("Open"=TRUE ("Open?")) -> (error out=w657:errorcluster)  [unwired: 3 in, 3 out]
            n279 = property on="Ctrl Tree" class="Tree (strict)"(error in=w657) -> ("All Tags"=w658:string[])  [unwired: 1 in, 2 out]
          }
          frame "Top-Level" {
            # "VI might have controls with non-unique names !"
            n280 = for {
              tunnel: w668 -> [w670] mode=indexing
              tunnel: [w669] -> w667 mode=indexing
              n281 = Unbundle By Name(w670) -> ("Ctrl ID"=w669:string)
            }
            n282 = Array Size(array=w664) -> (size(s)=w665:i32)
            n283 = Initialize Array("", w665) -> (w663:string[])
            n284 = for {
              tunnel: w664 -> [w679] mode=indexing
              tunnel: w667 -> [w678]
              shift-right: [w675] -> w661
              shift-left: w663 -> [w674]
              shift-right: [w672] -> w660
              shift-left: 0 -> [w673]
              n285 = Unbundle By Name(w679) -> ("Tree Tag"=w671:string, "Control ID"=w677:string)
              n286 = Search 1D Array(1D array=w678, element=w677) -> (index of element=w676:i32)  [unwired: 1 in]
              n287 = case shown="0.." w676 {
                tunnel: [w681 w685] -> w675
                tunnel: w674 -> [w681 w686]
                tunnel: w673 -> [w680 w684]
                tunnel: [w680 w683] -> w672
                tunnel: w671 -> [_ w682]
                frame ..-1 {
                }
                frame 0.. {
                  n288 = Increment(x=w684) -> (x+1=w683:i32)
                  n289 = Replace Array Subset(array=w686, new element=w682, index=w684) -> (w685:string[])
                }
              }
            }
            n290 = Reshape Array(w661, w660) -> (w659:string[])
          }
          frame "No Error" {
            n291 = property on="Ctrl Tree" class="Tree (strict)"() -> ("All Tags"=w689:string[])  [unwired: 2 in, 2 out]
            n292 = for {
              tunnel: w688 -> [w694] mode=indexing
              shift-right: [w691] -> w687
              shift-left: w689 -> [w693]
              n293 = Unbundle By Name(w694) -> ("Error Cluster"=w692:bool, "Tree Tag"=w690:string)
              n294 = case shown="True" w692 {
                tunnel: w693 -> [w695 w703]
                tunnel: w690 -> [_ w700]
                tunnel: [w695 w702] -> w691
                frame False {
                }
                frame True {
                  n295 = control-ref of="Ctrl Tree"() -> (w699:refnum<vi>)
                  n296 = call "VIH Project Tree - Get Tree Item Tags.vi"("Parent Item Tag"=w700, "Project Tree"=w699) -> ("Child Item Tags"=w697:string[], "dup Parent Item Tag"=w698:string)  [unwired: 6 in, 2 out]
                  n297 = Build Array (concatenate)(w698, w697) -> (w696:string[])
                  n298 = call "VIH Utility - STR - Filter 1D Array of Strings.vi"("Action (keep instances)"=enum16{"keep instances", "remove instances"}."remove instances", "instances"=w696, "Array in"=w703) -> ("Array out"=w702:string[])  [unwired: 7 in, 1 out]
                }
              }
            }
            n299 = for {
              tunnel: [w706] -> _
              tunnel: w687 -> [w704] mode=indexing
              n300 = invoke on="Ctrl Tree" class="Tree (strict)" method="Open/Close.Item"("tag"=w704, "Open"=TRUE ("Open?")) -> (error out=w706:errorcluster)  [unwired: 3 in, 4 out]
            }
          }
          frame "Error" {
            n301 = for {
              tunnel: w709 -> [w714] mode=indexing
              shift-right: [w711] -> w708
              shift-left: string[] [] ("Array out") -> [w713]
              n302 = Unbundle By Name(w714) -> ("Error Cluster"=w712:bool, "Tree Tag"=w710:string)
              n303 = case shown="True" w712 {
                tunnel: w713 -> [w715 w717]
                tunnel: w710 -> [_ w721]
                tunnel: [w715 w716] -> w711
                frame False {
                }
                frame True {
                  n304 = control-ref of="Ctrl Tree"() -> (w720:refnum<vi>)
                  n305 = call "VIH Project Tree - Get Tree Item Tags.vi"("Parent Item Tag"=w721, "Project Tree"=w720) -> ("Child Item Tags"=w718:string[], "dup Parent Item Tag"=w719:string)  [unwired: 6 in, 2 out]
                  n306 = Build Array (concatenate)(w717, w719, w718) -> (w716:string[])
                }
              }
            }
            n307 = for {
              tunnel: [w724] -> _
              tunnel: w708 -> [w722] mode=indexing
              n308 = invoke on="Ctrl Tree" class="Tree (strict)" method="Open/Close.Item"("tag"=w722, "Open"=TRUE ("Open?")) -> (error out=w724:errorcluster)  [unwired: 3 in, 4 out]
            }
          }
          frame "Enum & Ring" {
            n309 = for {
              tunnel: w727 -> [w732] mode=indexing
              shift-right: [w729] -> w726
              shift-left: string[] [] ("Array out") -> [w731]
              n310 = Unbundle By Name(w732) -> ("Class Name"=w730:string, "Tree Tag"=w728:string)
              n311 = case shown="\"Enum\", \"Ring\"" w730 {
                tunnel: w731 -> [w733 w736]
                tunnel: [w733 w735] -> w729
                tunnel: w728 -> [_ w734]
                frame Default {
                }
                frame "Enum", "Ring" {
                  n312 = Build Array (concatenate)(w736, w734) -> (w735:string[])
                }
              }
            }
            n313 = for {
              tunnel: [w739] -> _
              tunnel: w726 -> [w737] mode=indexing
              n314 = invoke on="Ctrl Tree" class="Tree (strict)" method="Open/Close.Item"("tag"=w737, "Open"=TRUE ("Open?")) -> (error out=w739:errorcluster)  [unwired: 3 in, 4 out]
            }
          }
          frame "Nested" {
            n315 = control-ref of="Ctrl Tree"() -> (w743:refnum<vi>)
            n316 = for {
              tunnel: w743 -> [w752]
              tunnel: w740 -> [w751] mode=indexing
              shift-right: [w747] -> w741
              shift-left: string[] [] -> [w748]
              n317 = call "VIH Project Tree - Get Tree Item Tags.vi"("Parent Item Tag"=w751, "Project Tree"=w752) -> ("Child Item Tags"=w749:string[], "dup Parent Item Tag"=w750:string)  [unwired: 6 in, 2 out]
              n318 = Build Array (concatenate)(w748, w750, w749) -> (w747:string[])
            }
            n319 = for {
              tunnel: [w746] -> _
              tunnel: w741 -> [w744] mode=indexing
              n320 = invoke on="Ctrl Tree" class="Tree (strict)" method="Open/Close.Item"("tag"=w744, "Open"=TRUE ("Open?")) -> (error out=w746:errorcluster)  [unwired: 3 in, 4 out]
            }
          }
        }
        n321 = property on="Ctrl Tree" class="Tree (strict)"("Value"=w652) -> ()  [unwired: 2 in, 2 out]
      }
    }
  }
  "dup VI Path" <- "VI Path"
